vi "Example.vi"() -> ()   [LabVIEW 2024]
uses:
  <vilib>/Utility/sysdir.llb/System Directory Type.ctl
  message with stats.ctl
  message.ctl
  message type.ctl
  message c2s.vi
  message with stats c2s.vi
  <vilib>/Utility/error.llb/Trim Whitespace.vi
  <vilib>/Utility/error.llb/Trim Whitespace One-Sided.vi
  atsj peakcan basic.lvlib
panel:
  in  "read delay":bool
  out "trace log entries":string
  out "summary":string
  out "current log dir":string
  out "current api version":string
  in  "controller index":u32
  out "error":errorcluster
  in  "stop":bool
  in  "ip address":string="192.168.1.1"
  # "(enable to see trace log entries)"
  # "implemented in api version 4.10.1.968"
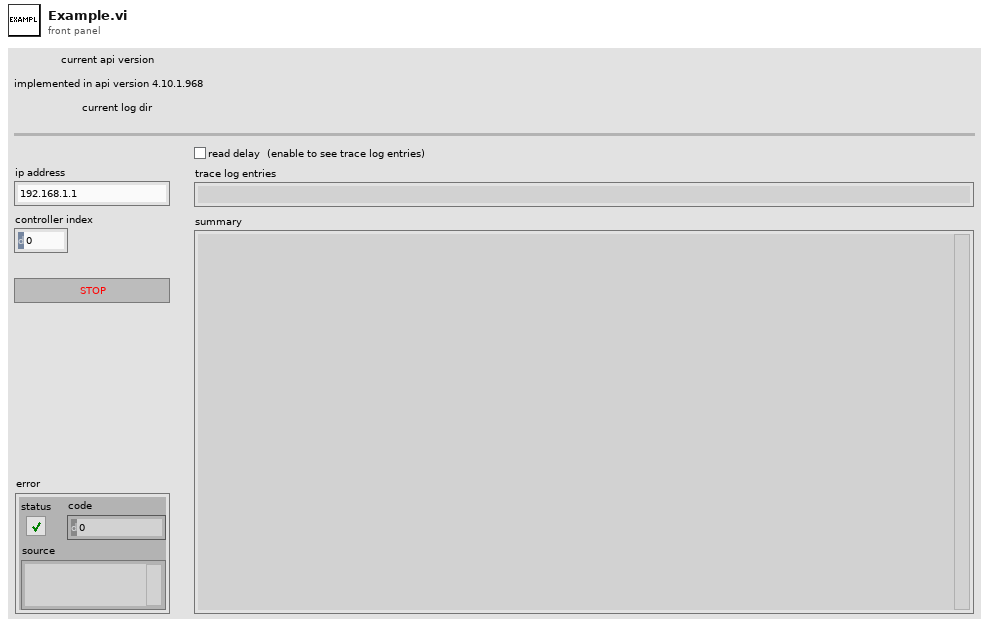
[diagram p1: front panel]
types:
  T1 = typedef "atsj peakcan basic.lvlib/message with stats.ctl" = cluster{"message":T2, "cycle time":u64, "count":u64}
  T2 = typedef "atsj peakcan basic.lvlib/message.ctl" = cluster{"id":u32, "message type":T3, "timestamp [us]":u64, "data":u8[]}
  T3 = typedef "atsj peakcan basic.lvlib/message type.ctl" = cluster{"remote transmission request ":bool, "extended":bool, "fd":bool, "fd bit rate switch":bool, "fd error state":bool, "echo":bool, "error":bool, "status":bool}
  T4 = typedef "System Directory Type.ctl" = i32
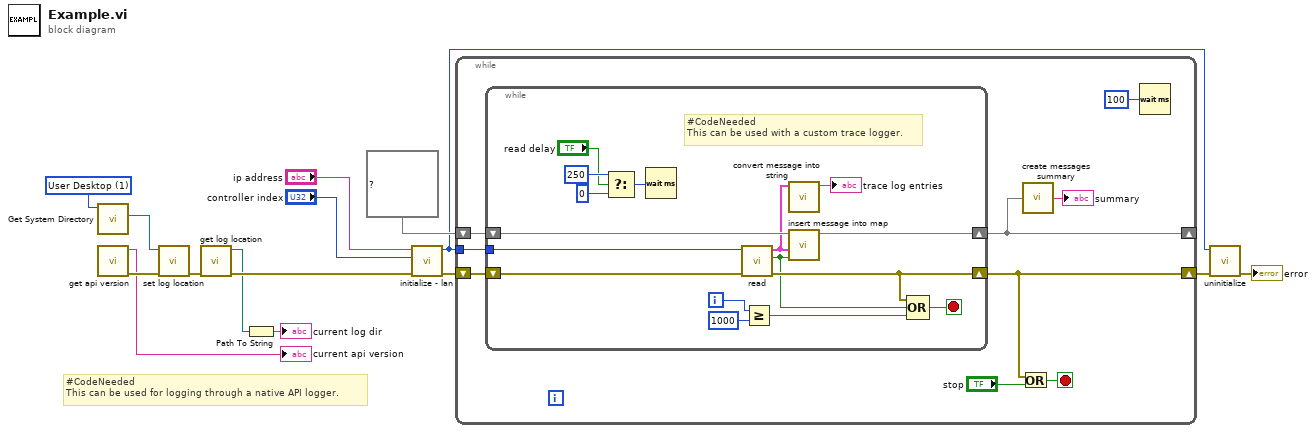
[diagram p0: block diagram]
diagram:
  w7 = T4 1 items=["User Home"=0, "User Desktop"=1, "User Documents"=2, "User Application Data"=3, "User Preferences"=4, "User Temporary"=5, "Public Documents"=6, "Public Application Data"=7, "Public Preferences"=8, "Public Cache"=13, "System Core Libraries"=9, "System Installed Libraries"=10, "Application Files"=11, "Boot Volume Root"=12] ("system directory type")
  # "#CodeNeeded\nThis can be used for logging through a native API logger."
  n1 = call <vilib>:"Get System Directory.vi"("system directory type"=w7) -> ("system directory"=w8:path)  [unwired: 10 in]
  n2 = call "get api version.vi"() -> ("error out"=w11:errorcluster, "api version"=→"current api version":string)  [unwired: 10 in]
  n3 = call "set log location.vi"("error in (no error)"=w11, "log directory"=w8) -> ("error out"=w10:errorcluster)  [unwired: 9 in]
  n4 = call "get log location.vi"("error in (no error)"=w10) -> ("error out"=w14:errorcluster, "log directory"=w6:path)  [unwired: 9 in]
  n5 = Path To String(path=w6) -> (string=→"current log dir":string)
  n6 = call "initialize - lan.vi"("error in (no error)"=w14, "controller index(0)"="controller index", "ip"="ip address") -> ("error out"=w1:errorcluster, "channel handle"=w4:u16)  [unwired: 7 in]
  n7 = while {
    shift-right: [w21] -> w13
    shift-left: w1 -> [w24]
    tunnel: w4 -> [w22]
    shift-right: [w17] -> _
    shift-left: map{u32, T1} {} ("messages out") -> [w18]
    stop <- w19 stop-if-true
    n8 = while {
      shift-right: [w36] -> w21
      shift-left: w24 -> [w40]
      tunnel: w22 -> [w39]
      shift-right: [w32] -> w17
      shift-left: w18 -> [w31]
      i -> [w38]
      stop <- w34 stop-if-true
      # "#CodeNeeded\nThis can be used with a custom trace logger."
      n9 = Select(t=u32 250, s="read delay", f=u32 0) -> (s? t:f=w27:u32)
      n10 = Wait (ms)(milliseconds to wait=w27) -> ()  [unwired: 1 out]
      n11 = call "read.vi"("error in (no error)"=w40, "channel handle"=w39) -> ("error out"=w36:errorcluster, "queue empty?"=w33:bool, "message"=w30:T2)  [unwired: 6 in, 1 out]
      n12 = Greater Or Equal?(x=w38, y=1000) -> (x >= y?=w35:bool)
      n13 = call "convert message into string.vi"("message"=w30) -> ("message string"=→"trace log entries":string)  [unwired: 7 in, 3 out]
      n14 = call "insert message into map.vi"("skip (F)"=w33, "message"=w30, "messages in"=w31) -> ("messages out"=w32:map{u32, T1})  [unwired: 8 in]
      n15 = Compound Arithmetic op=OR(w36, w33, w35) -> (w34:bool)
    }
    n16 = Or(x=w21, y="stop") -> (x .or. y?=w19:bool)
    n17 = call "create messages summary.vi"("messages map"=w17) -> ("messages summary"=→"summary":string)
    n18 = Wait (ms)(milliseconds to wait=u32 100) -> ()  [unwired: 1 out]
  }
  n19 = call "uninitialize.vi"("error in (no error)"=w13, "channel handle (0:all)"=w4) -> ("error out"=→"error":errorcluster)  [unwired: 9 in]
